vi "Connect Case Selector Terminal.vi"(8 "error in (no error)":errorcluster, 10 "Wire Source":refnum<vi>, 11 "Case Structure in":refnum<vi>) -> (0 "error IO":errorcluster, 3 "Case Structure out":refnum<vi>)   [LabVIEW 2019, in "gRPC Template Creation Utility.lvlib"]
uses:
  gRPC Template Creation Utility.lvlib
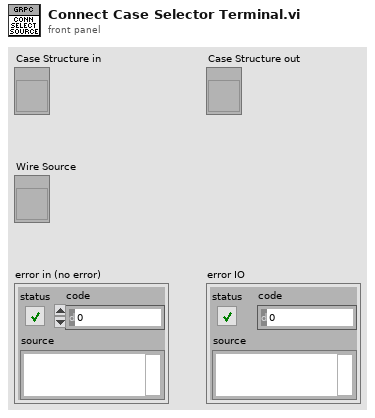
[diagram p1: front panel]
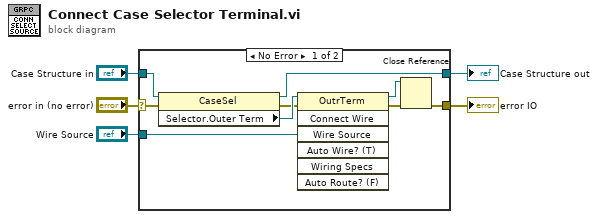
[diagram p0: block diagram]
diagram:
  n1 = case shown="No Error" "error in (no error)" {
    selector: "error in (no error)" -> [w10 w16]
    tunnel: "Case Structure in" -> [w12 w15]
    tunnel: [w11 w15] -> w3
    tunnel: [w7 w16] -> w2
    tunnel: "Wire Source" -> [w6 _]
    frame No Error {
      n2 = property class="CaseSel"(reference=w12, error in=w10) -> (reference out=w11:refnum<vi>, error out=w8:errorcluster, "Selector.Outer Term"=w9:refnum<vi>)
      n3 = invoke class="OutrTerm" method="Connect Wire"(reference=w9, error in=w8, "Wire Source"=w6) -> (reference out=w13:refnum<vi>, error out=w14:errorcluster)  [unwired: 4 in, 5 out]
      n4 = Close Reference(reference=w13, error in (no error)=w14) -> (error out=w7:errorcluster)
    }
    frame Error {
    }
  }
  "Case Structure out" <- w3
  "error IO" <- w2
